vi "DAC Save Results.vi"(8 "error in":errorcluster, 9 "Log Details?":bool, 10 "tdms file":refnum<k34>, 11 "DAC Pump Inv in":refnum<class "DAC Pump Inv.lvclass">) -> (0 "error out":errorcluster)   [LabVIEW 2019, in "DAC.lvlib" / "DAC Pump Inv.lvclass"]
uses:
  DAC Pump Inv.lvclass
  DAC.lvclass
  C:/Users/wg/Documents/LV_Projects/test-stand/App/DAC/DAC.lvclass
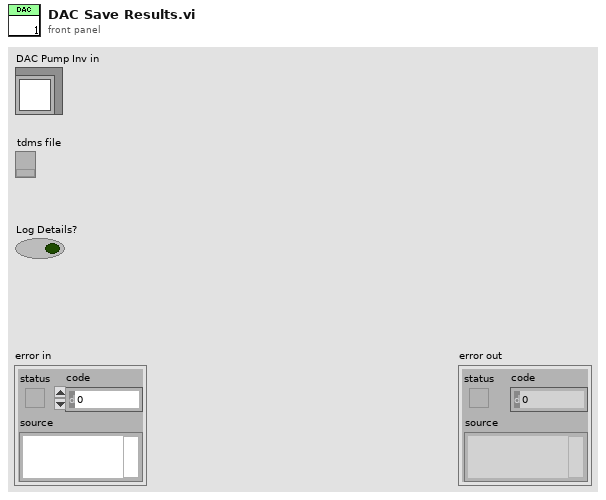
[diagram p1: front panel]
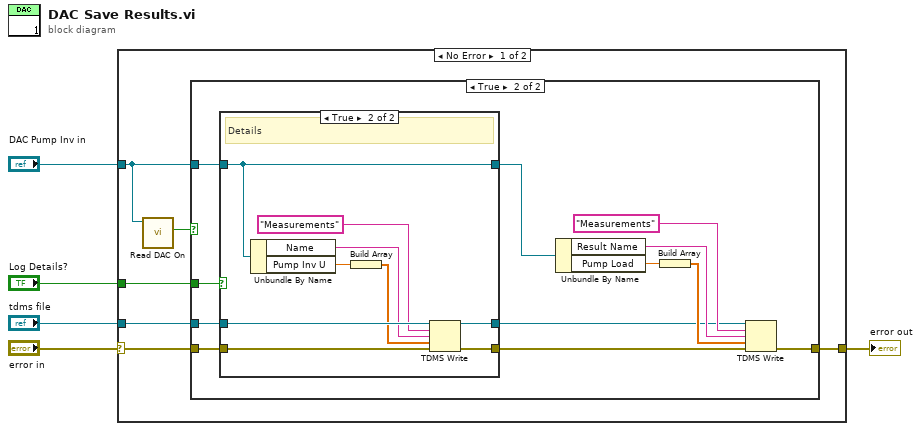
[diagram p0: block diagram]
diagram:
  n1 = case shown="No Error" "error in" {
    selector: "error in" -> [w8 w37]
    tunnel: "DAC Pump Inv in" -> [w11 _]
    tunnel: "tdms file" -> [w9 _]
    tunnel: [w7 w37] -> w3
    tunnel: "Log Details?" -> [w6 _]
    frame No Error {
      n2 = call "Read DAC On.vi"("DAC in"=w11) -> ("DAC On"=w10:bool)  [unwired: 8 in, 2 out]
      n3 = case shown="True" w10 {
        tunnel: w11 -> [_ w19]
        tunnel: w9 -> [_ w17]
        tunnel: w8 -> [w12 w16]
        tunnel: [w12 w20] -> w7
        tunnel: w6 -> [_ w15]
        frame False {
        }
        frame True {
          n4 = case shown="True" w15 {
            tunnel: w17 -> [w26 w36]
            tunnel: w16 -> [w27 w32]
            tunnel: w19 -> [w25 w29]
            tunnel: [w27 w31] -> w13
            tunnel: [w26 w30] -> w14
            tunnel: [w25 w29] -> w18
            frame False {
            }
            frame True {
              # "Details"
              n5 = Unbundle By Name(w29) -> ("Name"=w34:string, "Pump Inv U"=w28:dbl)
              n6 = Build Array(w28) -> (w35:dbl[])
              n7 = TDMS Write(0:w36, 5:"Measurements" ("group name in (Untitled)"), 7:w34, 9:w35, 11:w32) -> (4:w30:refnum<k34>, 15:w31:errorcluster)  [unwired: 1 in, 2 out]
            }
          }
          n8 = Unbundle By Name(w18) -> ("Result Name"=w22:string, "Pump Load"=w24:dbl)
          n9 = Build Array(w24) -> (w23:dbl[])
          n10 = TDMS Write(0:w14, 5:"Measurements" ("group name in (Untitled)"), 7:w22, 9:w23, 11:w13) -> (15:w20:errorcluster)  [unwired: 1 in, 3 out]
        }
      }
    }
    frame Error {
    }
  }
  "error out" <- w3
